vi "RDC-water-generate_calib_file.vi"(3 "Save Name":string, 5 "Save Path":path=path "C:/projects/VNA/src/LabVIEW/spike", 7 "LibreVNA samplerate file":path, 8 "Increment f (10MHz)":dbl=10000000.0, 9 "Stop f (6GHz) 2":dbl=6000000000.0, 10 "Start f (300MHz)":dbl=300000000.0, 11 "water Temp (25C) [10-40C]":dbl=25.0) -> (2 "Filepath":path)   [LabVIEW 2020, in "RDC-Reflection_Data_Computation.lvlib"]
doc: "Generates a water calibration file at the given water temperature (10-40 C), either over a frequency range or on the frequencies read from the LibreVNA samplerate file, and saves it with RFH-save-water_calib. Returns the file path."
uses:
  RDC-Reflection_Data_Computation.lvlib
  Reflector/RFH-common_data_format.ctl
  Reflector/RFH-Reflection_File_Handler.lvlib
panel:
  in  "Selector":bool
  out "status":string
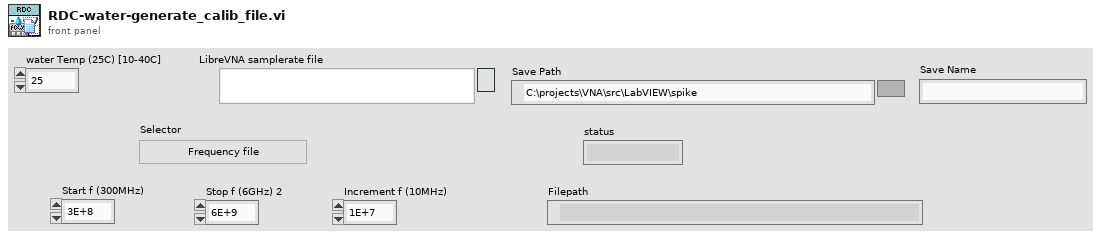
[diagram p1: front panel]
types:
  T1 = typedef "RFH-Reflection_File_Handler.lvlib/RFH-common_data_format.ctl" = cluster{"Frequency":dbl[], "Reflection'":dbl[], "Reflection''":dbl[], "Permativity'":dbl[], "Permativity''":dbl[], "Conductivity":dbl[], "Loss Tangent":dbl[], "Resistance":dbl[], "Reactance":dbl[]}
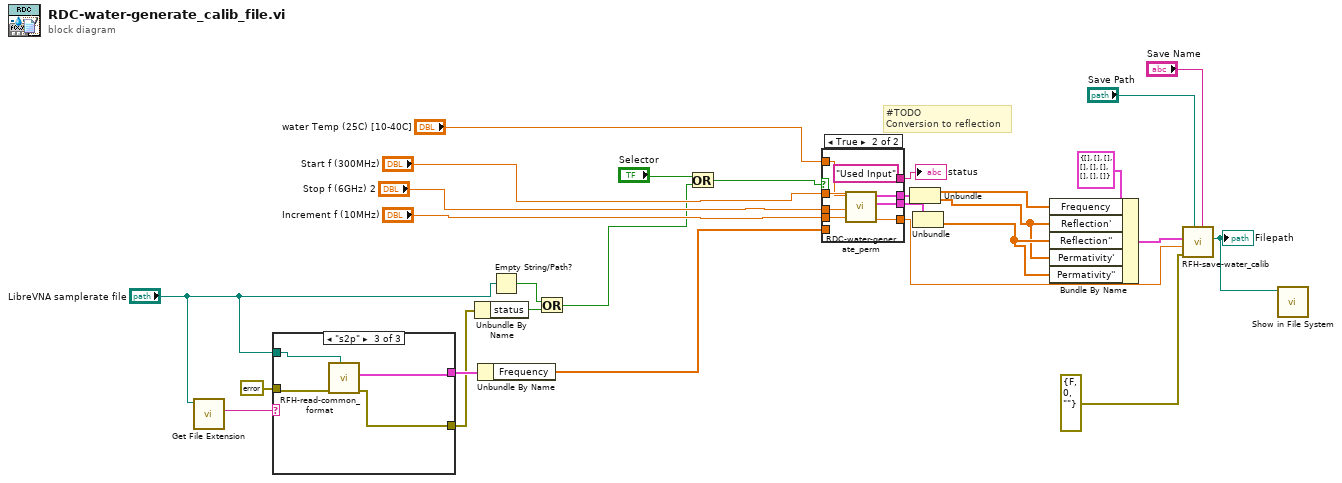
[diagram p0: block diagram]
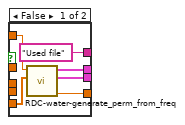
[diagram p2: hidden frame]
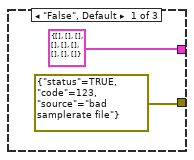
[diagram p3: hidden frame]
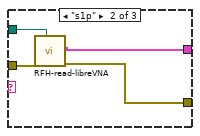
[diagram p4: hidden frame]
diagram:
  # "#TODO\nConversion to reflection"
  n1 = call <vilib>:"Get File Extension.vi"("file"="LibreVNA samplerate file") -> ("lowercase file extension"=w27:string)  [unwired: 6 in, 4 out]
  n2 = case shown="\"s2p\"" w27 {
    tunnel: [T1 {"Frequency"=[], "Reflection'"=[], "Reflection''"=[], "Permativity'"=[], "Permativity''"=[], "Conductivity"=[], "Loss Tangent"=[], "Resistance"=[], "Reactance"=[]} ("Common Format") w31 w37] -> w26
    tunnel: [errorcluster {"status"=TRUE, "code"=123, "source"="bad samplerate file"} ("error out") w32 w36] -> w22
    tunnel: errorcluster {"status"=FALSE, "code"=0, "source"=""} ("error out") -> [_ w33 w38]
    tunnel: "LibreVNA samplerate file" -> [_ w34 w35]
    frame "False", Default {
    }
    frame "s1p" {
      n3 = call "RFH-read-libreVNA.vi"("file path (dialog if empty)"=w34, "error in"=w33) -> ("error out"=w32:errorcluster, "Common Format"=w31:T1)  [unwired: 8 in]
    }
    frame "s2p" {
      n4 = call "RFH-read-common_format.vi"("file path (dialog if empty)"=w35, "error in"=w38) -> ("error out"=w36:errorcluster, "Common Format"=w37:T1)  [unwired: 8 in]
    }
  }
  n5 = Unbundle By Name(w22) -> ("status"=w21:bool)
  n6 = Unbundle By Name(w26) -> ("Frequency"=w4:dbl[])
  n7 = Empty String/Path?(string/path="LibreVNA samplerate file") -> (empty?=w19:bool)
  n8 = Or(x=w19, y=w21) -> (x .or. y?=w2:bool)
  n9 = Or(x="Selector", y=w2) -> (x .or. y?=w1:bool)
  n10 = case shown="True" w1 {
    tunnel: "Start f (300MHz)" -> [_ w52]
    tunnel: "Stop f (6GHz) 2" -> [_ w51]
    tunnel: "Increment f (10MHz)" -> [_ w50]
    tunnel: [w44 w49] -> w16
    tunnel: [w43 w48] -> w14
    tunnel: "water Temp (25C) [10-40C]" -> [w42 w47]
    tunnel: [w41 w46] -> w10
    tunnel: ["Used file" "Used Input"] -> w5
    tunnel: w4 -> [w39 _]
    frame False {
      n11 = call "RDC-water-generate_perm_from_freq.vi"("Frequency"=w39, "water Temp (25C) [10-40C]"=w42) -> ("used temp"=w41:dbl, "Imag Perm"=w43:cluster{dbl[], dbl[]}, "Real Perm"=w44:cluster{dbl[], dbl[]})  [unwired: 5 in, 2 out]
    }
    frame True {
      n12 = call "RDC-water-generate_perm.vi"("Increment f (10MHz)"=w50, "Stop f (6GHz) 2"=w51, "Start f (300MHz)"=w52, "water Temp (25C) [10-40C]"=w47) -> ("used temp"=w46:dbl, "Imag Perm"=w48:cluster{dbl[], dbl[]}, "Real Perm"=w49:cluster{dbl[], dbl[]})  [unwired: 3 in, 2 out]
    }
  }
  "status" <- w5
  n13 = Unbundle(w16) -> (w15:dbl[], w12:dbl[])
  n14 = Unbundle(w14) -> (w13:dbl[])  [unwired: 1 out]
  n15 = Bundle By Name(cluster=T1 {"Frequency"=[], "Reflection'"=[], "Reflection''"=[], "Permativity'"=[], "Permativity''"=[], "Conductivity"=[], "Loss Tangent"=[], "Resistance"=[], "Reactance"=[]} ("Common Format"), "Frequency"=w15, "Reflection'"=w12, "Reflection''"=w13, "Permativity'"=w12, "Permativity''"=w13) -> (w17:T1)
  n16 = call "RFH-save-water_calib.vi"("Save Name"="Save Name", "Save Path"="Save Path", "error in (no error)"=errorcluster {"status"=FALSE, "code"=0, "source"=""}, "Water temp"=w10, "Common Format"=w17) -> ("Filepath"=w7:path)  [unwired: 5 in, 1 out]
  "Filepath" <- w7
  n17 = call <vilib>:"Show in File System.vi"("file or directory path"=w7) -> ()  [unwired: 10 in, 1 out]
